vi "Set Control Label.vi"(2 "error in (no error)":errorcluster, 3 "Text":string, 4 "Control In":refnum<vi>) -> (0 "error out":errorcluster, 1 "Control Out":refnum<vi>)   [LabVIEW 2012, in "Scripting Tools.lvlib"]
doc: "Set the text of the label of the control referenced by <B>Control In</B>."
uses:
  Scripting Tools.lvlib
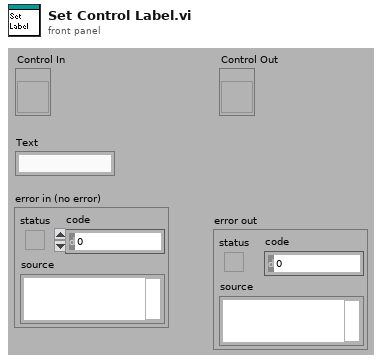
[diagram p1: front panel]
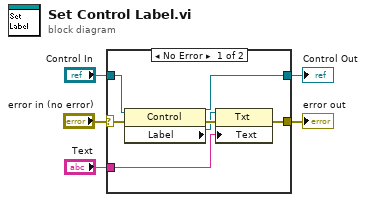
[diagram p0: block diagram]
diagram:
  n1 = case shown="No Error" "error in (no error)" {
    selector: "error in (no error)" -> [w7 w14]
    tunnel: "Control In" -> [w10 w13]
    tunnel: [w9 w13] -> w4
    tunnel: [w8 w14] -> w3
    tunnel: "Text" -> [w6 _]
    frame No Error {
      n2 = property class="Control"(reference=w10, error in=w7) -> (reference out=w9:refnum<vi>, error out=w12:errorcluster, "Label"=w11:refnum<vi>)
      n3 = property class="Txt"(reference=w11, error in=w12, "Text"=w6) -> (error out=w8:errorcluster)  [unwired: 1 out]
    }
    frame Error {
    }
  }
  "Control Out" <- w4
  "error out" <- w3
